vi "lvmcp_uid.vi"() -> ()   [LabVIEW 2026]
panel:
  out "error out":errorcluster
  out "UID":i32
  in  "reference":refnum<vi>
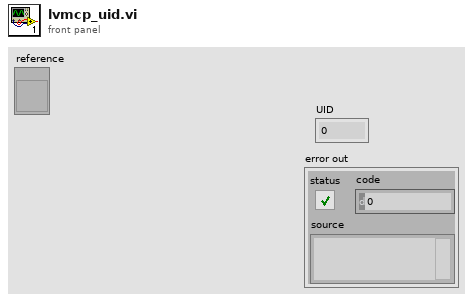
[diagram p1: front panel]
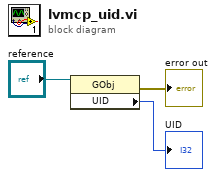
[diagram p0: block diagram]
diagram:
  n1 = property class="GObj"(reference="reference") -> (error out=→"error out":errorcluster, "UID"=→"UID":i32)  [unwired: 1 in, 1 out]
